vi "configuration UI.vi"() -> ()   [LabVIEW 2013, in "Tag Bus Web Interface editor node.lvclass"]
uses:
  Tag Bus Web Interface editor node.lvclass
  <vilib>/NI/Configuration Framework/Node/NodeRef.ctl
  <vilib>/NI/Configuration Framework/Node/NISE_CEF_Node.lvclass
  <vilib>/NI/AMC/Message Queue.ctl
  <vilib>/NI/AMC/Message.ctl
  <vilib>/NI/Tools/Keyed Array/KeyedArray.ctl
  <vilib>/NI/Configuration Framework/Node/UserEventRef.ctl
  <vilib>/NI/Configuration Framework/Controls/EventCluster.ctl
  Tag Bus Web Interface editor node.lvclass/Tag Bus Web Interface editor node.ctl
  <vilib>/NI/Configuration Framework/serializable configuration/NISE_CEF_serializable configuration.lvclass/NISE_CEF_serializable configuration.ctl
  <vilib>/NI/Tag Bus Module Framework/channel/channel classification.ctl
  <vilib>/NI/Tag Bus/tag/Data Type.ctl
  configuration/Tag Bus Web Interface configuration.lvclass
  <vilib>/NI/Tag Bus/tag/tag descriptor.lvclass/tag descriptor.ctl
  <vilib>/NI/Tag Bus/tag/read tag name.vi
  <vilib>/Utility/LVClass/Get LV Class Name.vi
  <vilib>/NI/Configuration Framework/error generator/NISE_error generator.vi
  <vilib>/NI/DCAF/Tag Editor Core/Configuration Editor/Classes/Engine Parent/read engine configuration.vi
  <vilib>/NI/DCAF/Tag Editor Core/Configuration Editor/Classes/Engine Parent/write engine configuration.vi
  <vilib>/NI/Module Execution Interface/Engine Configuration/engine configuration.lvclass
  <vilib>/NI/DCAF/Tag Editor Core/Configuration Editor/Classes/Module editor node/module editor node.lvclass
  <vilib>/NI/Configuration Framework/NISE_CEF_TreeControl.lvlib
  <vilib>/NI/Tag Bus/tag/tag descriptor.lvclass
  <vilib>/NI/Tag Bus Module Framework/channel/TBM channel.lvclass
  <vilib>/NI/DCAF/Tag Editor Core/Configuration Editor/Classes/Engine Parent/Engine Parent Editor Node.lvclass
  <vilib>/NI/Configuration Framework/serializable configuration/NISE_CEF_serializable configuration.lvclass
  <vilib>/NI/Tools/Keyed Array/Tools_KeyedArray.lvlib
  <vilib>/NI/AMC/AMC.lvlib
panel:
  in  "Tab Control":enum32{"Web Configuration"}(tab)
  in  "remove to":bool
  in  "add to":bool
  in  "remove from":bool
  in  "add from":bool
  in  "toTBWlist":i32(listbox)
  in  "fromTBWlist":i32(listbox)
  in  "avail tags":i32(listbox)=-1
  in  "Direction":enum32{"From TBWI", "To TBWI"}(radio)
  in  "user event":T1
  in  "main queue":T2
  in  "node ref":T3
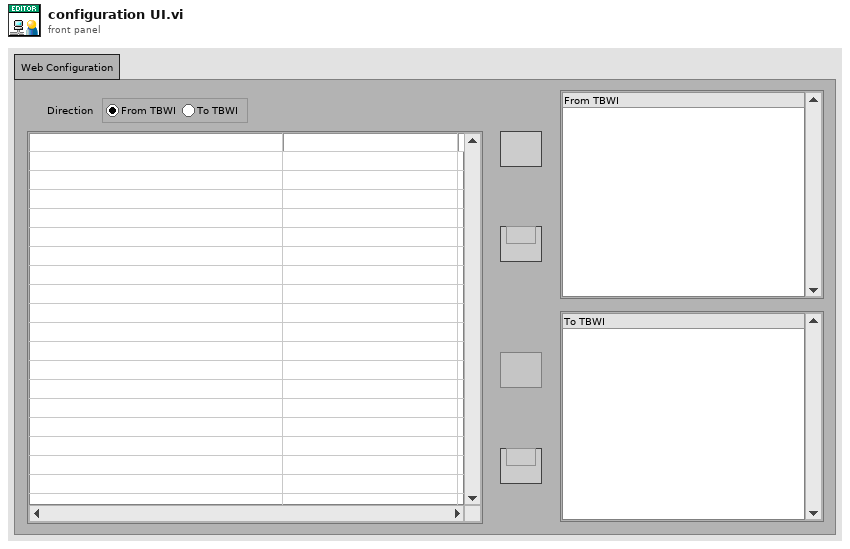
[diagram p1: front panel]
types:
  T1 = typedef "NISE_CEF_Node.lvclass/UserEventRef.ctl" = refnum<user-event>
  T2 = typedef "AMC.lvlib/Message Queue.ctl" = refnum<queue>
  T3 = typedef "NISE_CEF_Node.lvclass/NodeRef.ctl" = refnum<data-value>
  T4 = typedef "NISE_CEF_TreeControl.lvlib/EventCluster.ctl" = cluster{"command":string, "data":string}
  T5 = enum8{"Enabled", "Disabled", "Disabled and Grayed Out"}
  T6 = typedef "tag bus.lvlib/tag descriptor.lvclass/Data Type.ctl" = enum16{"Double", "Single", "I64", "I32", "I16", "I8", "U64", "U32", "U16", "U8", "Boolean", "String", "Array of Double", "Array of Single", "Array of I64", "Array of I32", "Array of I16", "Array of I8", "Array of U64", "Array of U32", "Array of U16", "Array of U8", "Array of Boolean", "Array of String"}
  T7 = typedef "TBM channel.lvclass/channel classification.ctl" = enum16{"input data", "output data", "processing parameter", "processing result"}
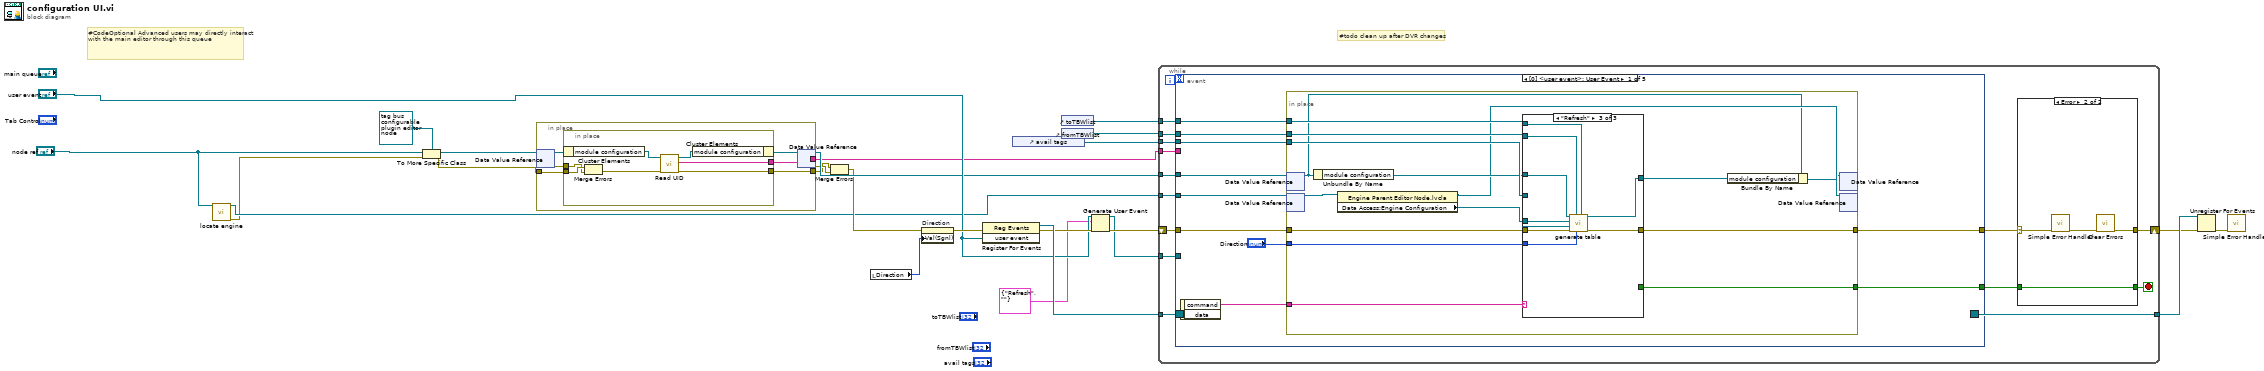
[diagram p0: block diagram]
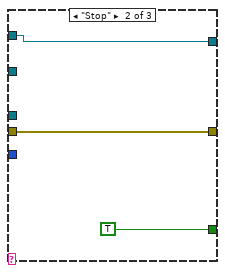
[diagram p4: hidden frame]
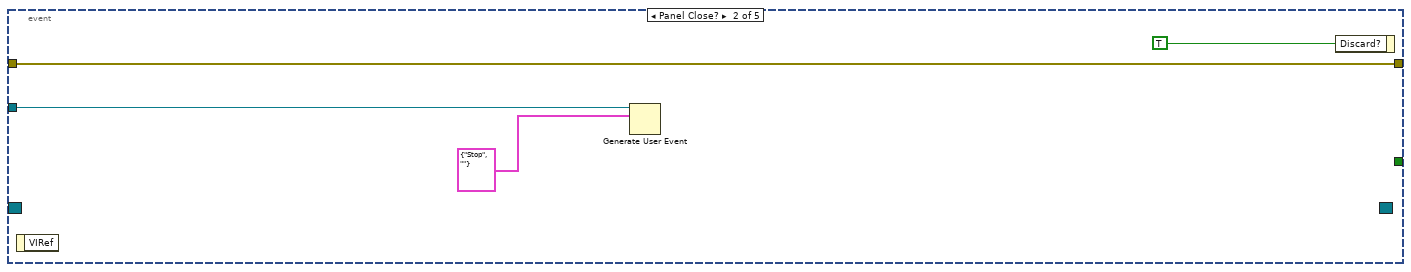
[diagram p5: hidden frame]
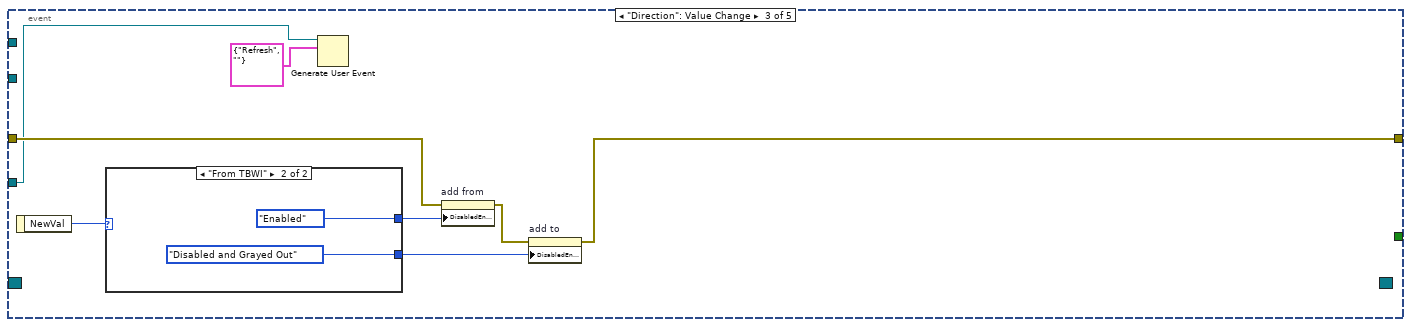
[diagram p6: hidden frame]
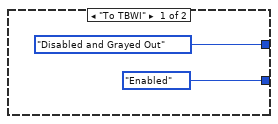
[diagram p7: hidden frame]
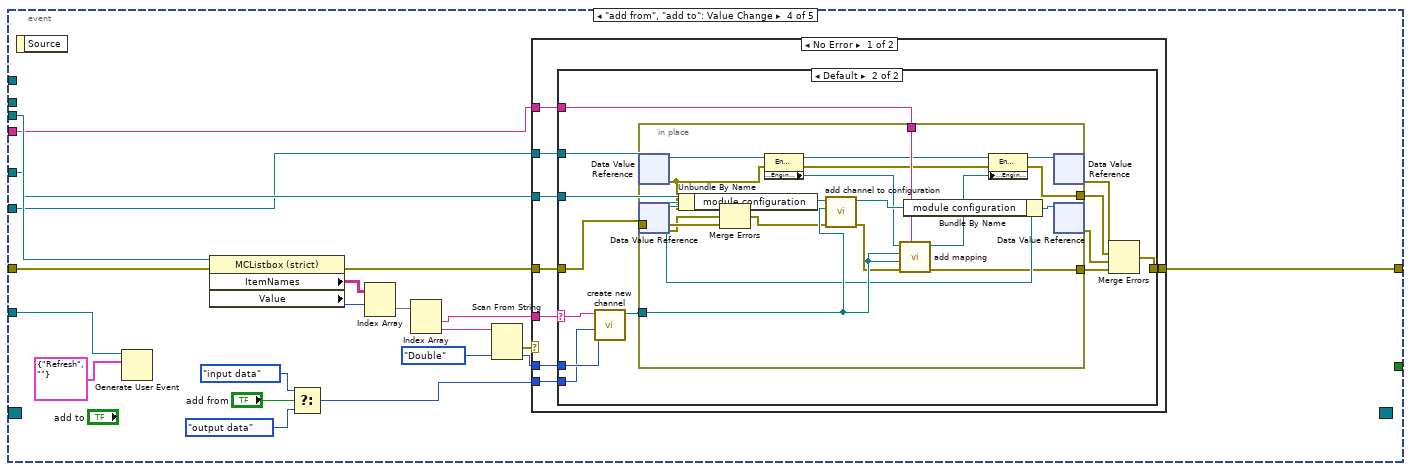
[diagram p8: hidden frame]
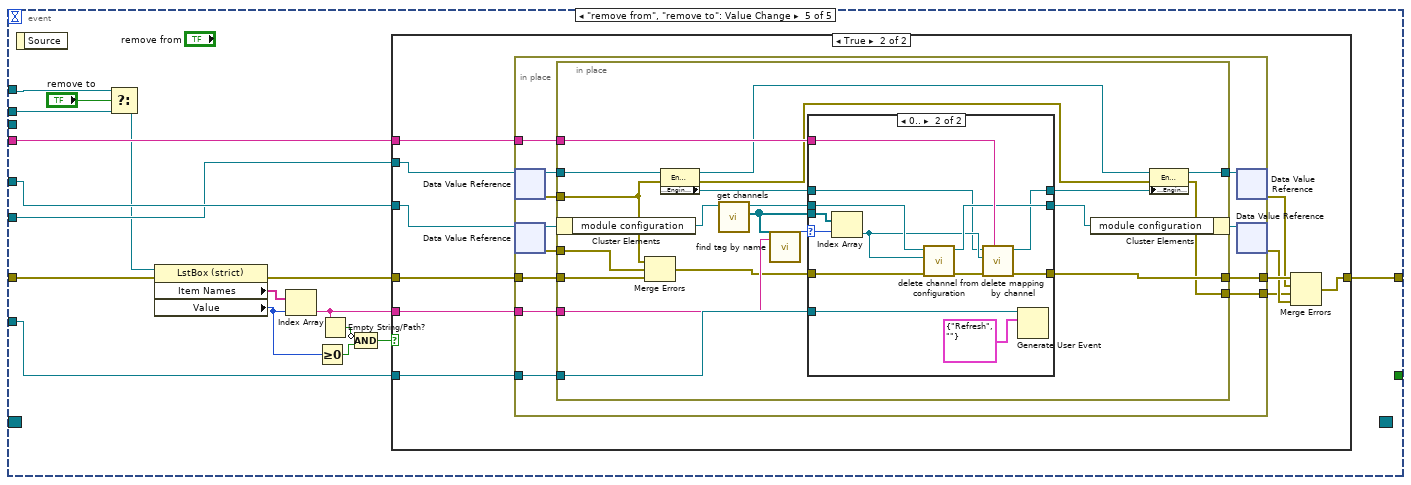
[diagram p11: hidden frame]
diagram:
  # "#todo clean up after DVR changes"
  # "#CodeOptional Advanced users may directly interact with the main editor through this queue"
  n1 = call <vilib>:"locate engine.vi"("component"="node ref") -> ("error out"=w1:errorcluster, "engine"=w2:refnum<data-value>)  [unwired: 9 in]
  n2 = To More Specific Class(target class=refnum<data-value> refnum ("data value reference"), reference="node ref", error in=w1) -> (specific class reference=w10:refnum<data-value>, error out=w8:errorcluster)
  n3 = in-place {
    in-place-border: w8 -> [w29]
    in-place-border: [w28] -> w6
    in-place-border: [w27] -> w5
    n4 = in-place-dvr #1(w10) -> (w31:refnum<class "Tag Bus Web Interface editor node.lvclass">, w30:errorcluster)
    n5 = in-place {
      in-place-border: w30 -> [w37]
      in-place-border: w29 -> [w38]
      in-place-border: [w33] -> w28
      in-place-border: [w32] -> w27
      n6 = in-place-cluster #2(w31) -> ("module configuration"=w36:refnum<class "Tag Bus Web Interface configuration.lvclass">)
      n7 = Merge Errors(w38, w37) -> (w34:errorcluster)
      n8 = call <vilib>:"Read UID.vi"("error in"=w34, "configuration in"=w36) -> ("error out"=w33:errorcluster, "instance id"=w32:string, "configuration out"=w35:refnum<class "Tag Bus Web Interface configuration.lvclass">)  [unwired: 7 in]
      n9 = in-place-cluster #2("module configuration"=w35) -> (w26:refnum<class "Tag Bus Web Interface editor node.lvclass">)
    }
    n10 = in-place-dvr #1(w26) -> (w9:refnum<data-value>, w7:errorcluster)
  }
  n11 = Merge Errors(w6, w7) -> (w4:errorcluster)
  n12 = local read "Direction"() -> (w15:enum32{"From TBWI", "To TBWI"})
  n13 = property on="Direction" class="RadioBtnsControl (strict)"(error in=w4, "Val(Sgnl)"=w15) -> (error out=w16:errorcluster)  [unwired: 1 in, 1 out]
  n14 = register-events(error in=w16, "user event") -> (reference out=w25:refnum<event-registration>, error out=w21:errorcluster)  [unwired: 1 in]
  n15 = control-ref of="avail tags"() -> (w19:refnum<vi>)
  n16 = control-ref of="toTBWlist"() -> (w18:refnum<vi>)
  n17 = control-ref of="fromTBWlist"() -> (w17:refnum<vi>)
  n18 = Generate User Event(user event="user event", event data cluster=T4 {"command"="Refresh", "data"=""} ("event data"), error in=w21) -> (user event out=w12:T1, error out=w14:errorcluster)  [unwired: 1 in]
  n19 = while {
    tunnel: w25 -> [w52]
    tunnel: [w51] -> w24
    shift-right: [w47] -> w23
    shift-left: w14 -> [w50]
    tunnel: w5 -> [w44]
    tunnel: w19 -> [w42]
    tunnel: w12 -> [w41]
    tunnel: w18 -> [w40]
    tunnel: w17 -> [w39]
    tunnel: w9 -> [w46]
    tunnel: w2 -> [w45]
    stop <- w49 stop-if-true
    n20 = event shown="[0] <user event>: User Event" {
      selector: w52 -> [_ _ _ _ _]
      dyn-events: [_ _ _ _ _] -> w51
      timeout: _ -> [_ _ _ _ _]
      tunnel: [w68 _ _ _ _] -> w48
      tunnel: [w66 w101 w104 w115 w183] -> w43
      tunnel: w50 -> [w65 w101 w105 w120 w178]
      tunnel: w46 -> [w60 _ _ w118 w182]
      tunnel: w45 -> [w59 _ _ w117 w181]
      tunnel: w44 -> [_ _ _ w116 w180]
      tunnel: w42 -> [w64 _ _ w119 _]
      tunnel: w41 -> [_ w99 w102 w134 w177]
      tunnel: w40 -> [w62 _ _ _ w193]
      tunnel: w39 -> [w63 _ _ _ w191]
      event User Event {
        n21 = event-data() -> ("command"=w67:string)  [unwired: 1 in, 1 out]
        n22 = in-place {
          in-place-border: [w83] -> w68
          in-place-border: w67 -> [w82]
          in-place-border: [w81] -> w66
          in-place-border: w65 -> [w80]
          in-place-border: w64 -> [w79]
          in-place-border: w63 -> [w78]
          in-place-border: w62 -> [w77]
          in-place-border: "Direction" -> [w76]
          n23 = in-place-dvr #3(w60) -> (w71:refnum<class "Tag Bus Web Interface editor node.lvclass">)  [unwired: 1 out]
          n24 = in-place-dvr #4(w59) -> (w75:refnum<class "Engine Parent Editor Node.lvclass">)  [unwired: 1 out]
          n25 = Unbundle By Name(w71) -> ("module configuration"=w74:refnum<class "Tag Bus Web Interface configuration.lvclass">)
          n26 = property class="Engine Parent Editor Node.lvcla"(reference=w75) -> (reference out=w72:refnum<class "Engine Parent Editor Node.lvclass">, "Data Access:Engine Configuration"=w73:refnum<class "engine configuration.lvclass">)  [unwired: 1 in, 1 out]
          n27 = case shown="\"Refresh\"" w82 {
            tunnel: [_ TRUE _] -> w83
            tunnel: [w85 w87 w96] -> w81
            tunnel: w80 -> [w85 w87 w97]
            tunnel: w79 -> [_ _ w92]
            tunnel: w78 -> [_ _ w95]
            tunnel: w77 -> [_ _ w94]
            tunnel: w76 -> [_ _ w93]
            tunnel: w74 -> [w84 w86 w90]
            tunnel: w73 -> [_ _ w89]
            tunnel: [w84 w86 w91] -> w70
            frame Default {
            }
            frame "Stop" {
            }
            frame "Refresh" {
              n28 = call "generate table.vi"("to tbwi"=w94, "Direction"=w93, "from tbwi"=w95, "error in"=w97, "tags"=w92, "engine configuration in"=w89, "Tag Bus Web Interface configuration in"=w90) -> ("error out"=w96:errorcluster, "TBWI Cfg out"=w91:refnum<class "Tag Bus Web Interface configuration.lvclass">)  [unwired: 3 in]
            }
          }
          n29 = Bundle By Name(cluster=w71, "module configuration"=w70) -> (w69:refnum<class "Tag Bus Web Interface editor node.lvclass">)
          n30 = in-place-dvr #3(w69) -> ()  [unwired: 2 out]
          n31 = in-place-dvr #4(w72) -> ()  [unwired: 2 out]
        }
      }
      event Panel Close? {
        n32 = event-data() -> ()  [unwired: 1 in, 1 out]
        n33 = Generate User Event(user event=w99, event data cluster=T4 {"command"="Stop", "data"=""} ("event data")) -> ()  [unwired: 2 in, 2 out]
        n34 = event-data("Discard?"=TRUE) -> ()  [unwired: 1 in, 1 out]
      }
      event "Direction": Value Change {
        n35 = event-data() -> ("NewVal"=w109:enum32{"From TBWI", "To TBWI"})  [unwired: 1 in]
        n36 = case shown="\"From TBWI\"" w109 {
          tunnel: [T5."Disabled and Grayed Out" ("Disabled") T5."Enabled" ("Disabled")] -> w108
          tunnel: [T5."Enabled" ("Disabled") T5."Disabled and Grayed Out" ("Disabled")] -> w107
          frame "To TBWI" {
          }
          frame "From TBWI" {
          }
        }
        n37 = Generate User Event(user event=w102, event data cluster=T4 {"command"="Refresh", "data"=""} ("event data")) -> ()  [unwired: 2 in, 2 out]
        n38 = property on="add from" class="Bool"(error in=w105, "DisabledEnum"=w108) -> (error out=w106:errorcluster)  [unwired: 1 in, 1 out]
        n39 = property on="add to" class="Bool"(error in=w106, "DisabledEnum"=w107) -> (error out=w104:errorcluster)  [unwired: 1 in, 1 out]
      }
      event "add from", "add to": Value Change {
        n40 = event-data() -> ()  [unwired: 1 in, 1 out]
        n41 = Generate User Event(user event=w134, event data cluster=T4 {"command"="Refresh", "data"=""} ("event data")) -> ()  [unwired: 2 in, 2 out]
        n42 = property class="MCListbox (strict)"(reference=w119, error in=w120) -> (error out=w121:errorcluster, "ItemNames"=w122:string[][], "Value"=w123:i32)  [unwired: 1 out]
        n43 = Select(t=channel_classification."input data" ("channel classification"), s="add from", f=channel_classification."output data" ("channel classification")) -> (s? t:f=w114:T7)
        n44 = Index Array(array=w122, index (row)=w123) -> (element=w126:string[])  [unwired: 1 in]
        n45 = Index Array(array=w126) -> (element #1=w127:string, element #2=w124:string)  [unwired: 2 in]
        n46 = Scan From String(input string=w124, default 1=Data_Type."Double" ("data type")) -> (error out=w128:errorcluster, output 1=w129:T6)  [unwired: 3 in, 2 out]
        n47 = case shown="No Error" w128 {
          tunnel: [w142 w176] -> w115
          tunnel: w116 -> [w141 _]
          tunnel: w118 -> [w140 _]
          tunnel: w117 -> [w139 _]
          tunnel: w121 -> [w138 w176]
          tunnel: w127 -> [w137 _]
          tunnel: w129 -> [w136 _]
          tunnel: w114 -> [w135 _]
          frame No Error {
            n48 = case shown="Default" w137 {
              selector: w137 -> [_ w154]
              tunnel: [w143 w148] -> w142
              tunnel: w138 -> [w143 w156]
              tunnel: w139 -> [_ w149]
              tunnel: w140 -> [_ w150]
              tunnel: w141 -> [_ w155]
              tunnel: w136 -> [_ w153]
              tunnel: w135 -> [_ w151]
              frame "" {
              }
              frame Default {
                n49 = call <vilib>:"create new channel.vi"("channel classification"=w151, "data type"=w153, "channel name"=w154) -> ("channel"=w152:refnum<class "TBM channel.lvclass">)  [unwired: 8 in]
                n50 = in-place {
                  in-place-border: w156 -> [w175]
                  in-place-border: w155 -> [w174]
                  in-place-border: w152 -> [w173]
                  in-place-border: [w161] -> w145
                  in-place-border: [w157] -> w144
                  n51 = in-place-dvr #5(w149) -> (w167:refnum<class "Engine Parent Editor Node.lvclass">, w158:errorcluster)
                  n52 = in-place-dvr #6(w150) -> (w170:refnum<class "Tag Bus Web Interface editor node.lvclass">, w162:errorcluster)
                  n53 = Unbundle By Name(w170) -> ("module configuration"=w171:refnum<class "Tag Bus Web Interface configuration.lvclass">)
                  n54 = Merge Errors(w158, w162, w175) -> (w160:errorcluster)
                  n55 = property class="Engine Parent Editor Node.lvcla"(reference=w167, error in=w158) -> (reference out=w166:refnum<class "Engine Parent Editor Node.lvclass">, error out=w159:errorcluster, "Data Access:Engine Configuration"=w164:refnum<class "engine configuration.lvclass">)
                  n56 = call "add channel to configuration.vi"("error in"=w160, "TBM channel in"=w173, "Tag Bus Web Interface configuration in"=w171) -> ("error out"=w172:errorcluster, "Tag Bus Web Interface configuration out"=w168:refnum<class "Tag Bus Web Interface configuration.lvclass">)  [unwired: 7 in]
                  n57 = call <vilib>:"add mapping.vi"("owner ID"=w174, "error in"=w172, "channel"=w173, "tag descriptor"=w173, "engine configuration"=w164) -> ("error out"=w161:errorcluster, "engine configuration out"=w165:refnum<class "engine configuration.lvclass">)  [unwired: 5 in]
                  n58 = Bundle By Name(cluster=w170, "module configuration"=w168) -> (w169:refnum<class "Tag Bus Web Interface editor node.lvclass">)
                  n59 = property class="Engine Parent Editor Node.lvcla"(reference=w166, error in=w159, "Data Access:Engine Configuration"=w165) -> (reference out=w163:refnum<class "Engine Parent Editor Node.lvclass">, error out=w157:errorcluster)
                  n60 = in-place-dvr #5(w163) -> (w147:errorcluster)  [unwired: 1 out]
                  n61 = in-place-dvr #6(w169) -> (w146:errorcluster)  [unwired: 1 out]
                }
                n62 = Merge Errors(w147, w144, w146, w145) -> (w148:errorcluster)
              }
            }
          }
          frame Error {
          }
        }
      }
      event "remove from", "remove to": Value Change {
        n63 = event-data() -> ()  [unwired: 1 in, 1 out]
        n64 = Select(t=w193, s="remove to", f=w191) -> (s? t:f=w179:refnum<vi>)
        n65 = property class="LstBox (strict)"(reference=w179, error in=w178) -> (error out=w189:errorcluster, "Item Names"=w184:string[], "Value"=w185:i32)  [unwired: 1 out]
        n66 = Index Array(array=w184, index=w185) -> (element=w190:string)
        n67 = Greater Or Equal To 0?(x=w185) -> (x >= 0?=w187:bool)
        n68 = Empty String/Path?(string/path=w190) -> (empty?=w186:bool)
        n69 = Compound Arithmetic op=AND(invert w186, w187) -> (w188:bool)
        n70 = case shown="True" w188 {
          tunnel: w189 -> [w194 w202]
          tunnel: [w194 w198] -> w183
          tunnel: w182 -> [_ w200]
          tunnel: w181 -> [_ w199]
          tunnel: w177 -> [_ w205]
          tunnel: w190 -> [_ w204]
          tunnel: w180 -> [_ w201]
          frame False {
          }
          frame True {
            n71 = in-place {
              in-place-border: w205 -> [w217]
              in-place-border: w204 -> [w216]
              in-place-border: [w215] -> w203
              in-place-border: w202 -> [w214]
              in-place-border: w201 -> [w213]
              in-place-border: [w206] -> w195
              n72 = in-place-dvr #7(w199) -> (w208:refnum<class "Engine Parent Editor Node.lvclass">, w210:errorcluster)
              n73 = in-place-dvr #8(w200) -> (w212:refnum<class "Tag Bus Web Interface editor node.lvclass">, w209:errorcluster)
              n74 = in-place {
                in-place-border: w217 -> [w237]
                in-place-border: w216 -> [w236]
                in-place-border: [w233] -> w215
                in-place-border: w214 -> [w232]
                in-place-border: w213 -> [w230]
                in-place-border: w210 -> [w218]
                in-place-border: w209 -> [w226]
                in-place-border: w208 -> [w225]
                in-place-border: [w224] -> w207
                in-place-border: [w220] -> w206
                n75 = in-place-cluster #9(w212) -> ("module configuration"=w228:refnum<class "Tag Bus Web Interface configuration.lvclass">)
                n76 = Merge Errors(w218, w226, w232) -> (w227:errorcluster)
                n77 = property class="Engine Parent Editor Node.lvcla"(reference=w225, error in=w218) -> (reference out=w223:refnum<class "Engine Parent Editor Node.lvclass">, error out=w219:errorcluster, "Data Access:Engine Configuration"=w222:refnum<class "engine configuration.lvclass">)
                n78 = call-dynamic "get channels.vi"("Tag Bus Web Interface configuration in"=w228) -> ("channels"=w231:refnum<class "TBM channel.lvclass">[], "Tag Bus Web Interface configuration out"=w234:refnum<class "Tag Bus Web Interface configuration.lvclass">)  [unwired: 9 in]
                n79 = call <vilib>:"find tag by name.vi"("name"=w236, "tags in"=w231) -> ("index"=w235:i32)  [unwired: 9 in]
                n80 = case shown="0.." w235 {
                  selector: w235 -> [_ w251]
                  tunnel: w237 -> [_ w252]
                  tunnel: w234 -> [w240 w249]
                  tunnel: [w240 w245] -> w229
                  tunnel: [w239 w244] -> w233
                  tunnel: w227 -> [w239 w248]
                  tunnel: w231 -> [_ w250]
                  tunnel: w230 -> [_ w246]
                  tunnel: w222 -> [w238 w242]
                  tunnel: [w238 w241] -> w221
                  frame ..-1 {
                  }
                  frame 0.. {
                    n81 = Index Array(array=w250, index=w251) -> (element=w243:refnum<class "TBM channel.lvclass">)
                    n82 = call "delete channel from configuration.vi"("error in"=w248, "TBM channel in"=w243, "Tag Bus Web Interface configuration in"=w249) -> ("error out"=w247:errorcluster, "Tag Bus Web Interface configuration out"=w245:refnum<class "Tag Bus Web Interface configuration.lvclass">)  [unwired: 7 in]
                    n83 = call <vilib>:"delete mapping by channel.vi"("owner ID"=w246, "error in"=w247, "channel"=w243, "engine configuration in"=w242) -> ("error out"=w244:errorcluster, "engine configuration out"=w241:refnum<class "engine configuration.lvclass">)  [unwired: 6 in]
                    n84 = Generate User Event(user event=w252, event data cluster=T4 {"command"="Refresh", "data"=""} ("event data")) -> ()  [unwired: 2 in, 2 out]
                  }
                }
                n85 = in-place-cluster #9("module configuration"=w229) -> (w211:refnum<class "Tag Bus Web Interface editor node.lvclass">)
                n86 = property class="Engine Parent Editor Node.lvcla"(reference=w223, error in=w219, "Data Access:Engine Configuration"=w221) -> (reference out=w224:refnum<class "Engine Parent Editor Node.lvclass">, error out=w220:errorcluster)
              }
              n87 = in-place-dvr #7(w207) -> (w197:errorcluster)  [unwired: 1 out]
              n88 = in-place-dvr #8(w211) -> (w196:errorcluster)  [unwired: 1 out]
            }
            n89 = Merge Errors(w203, w197, w195, w196) -> (w198:errorcluster)
          }
        }
      }
    }
    n90 = case shown="Error" w43 {
      selector: w43 -> [w53 w57]
      tunnel: [w54 w58] -> w49
      tunnel: w48 -> [w54 w58]
      tunnel: [w53 w55] -> w47
      frame No Error {
      }
      frame Error {
        n91 = call <vilib>:"Simple Error Handler.vi"("error in (no error)"=w57) -> ("error out"=w56:errorcluster)  [unwired: 4 in, 4 out]
        n92 = call <vilib>:"Clear Errors.vi"("error in (no error)"=w56) -> ("error out"=w55:errorcluster)  [unwired: 6 in]
      }
    }
  }
  n93 = Unregister For Events(event registration refnum=w24, error in=w23) -> (error out=w20:errorcluster)
  n94 = call <vilib>:"Simple Error Handler.vi"("error in (no error)"=w20) -> ()  [unwired: 4 in, 5 out]
